vi "Empty-Arr.vi"(11 "数组 2":string[](array[string])=["1", "2", "3", "4"]) -> (3 "数组":string[](array[string]))   [LabVIEW 2025]
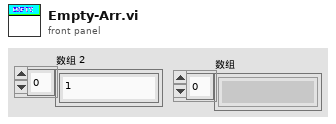
[diagram p1: front panel]
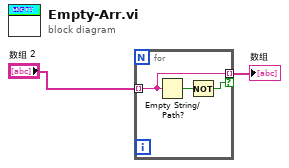
[diagram p0: block diagram]
diagram:
  n1 = for {
    tunnel: "数组 2" -> [w5] mode=indexing
    tunnel: [w5] -> w2 mode=indexing if=w3
    n2 = Empty String/Path?(string/path=w5) -> (empty?=w4:bool)
    n3 = Not(x=w4) -> (.not. x?=w3:bool)
  }
  "数组" <- w2
